vi "SetValueByArrayName.vi"(0 "VI Reference In":refnum<vi>, 2 "delimiter (>>)":string=">>", 5 "Control Path":string, 7 "Name Array":T1[](array[typedef]), 11 "Error In":errorcluster) -> (4 "VI Reference Out":refnum<vi>, 15 "Error Out":errorcluster)   [LabVIEW 2016, in "Drona.lvlib" / "ControlValue.lvlib" / "StimulusListbox.lvlib"]
doc: "Sets value(signaling) for the multi select listbox control whose item names with its occurrence are specified. Set the value as 1 in occurrence to select the first occurrence of an item. \n\nThe input control name is given as a string , incase of path, use delimiters inbetween the path."
uses:
  StimulusListbox.lvlib
  typedef/Name&Occurrence.ctl
  <userlib>/_OpenG.lib/array/array.llb/Search 1D Array (String)__ogtk.vi
  <vilib>/Utility/error.llb/Error Cluster From Error Code.vi
  <vilib>/ErrorRing/Error Ring.xnode
  Drona.lvlib
  Get/GetControlRef/GetControlRef.lvlib
  ControlValue.lvlib
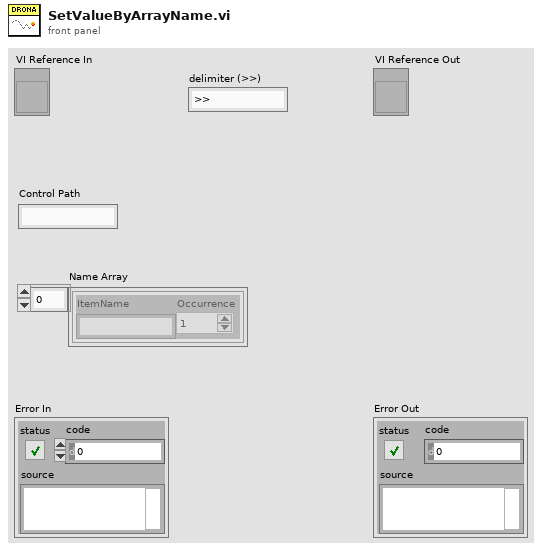
[diagram p1: front panel]
types:
  T1 = typedef "Drona.lvlib/ControlValue.lvlib/Name&Occurrence.ctl" = cluster{"ItemName":string, "Occurrence":i32}
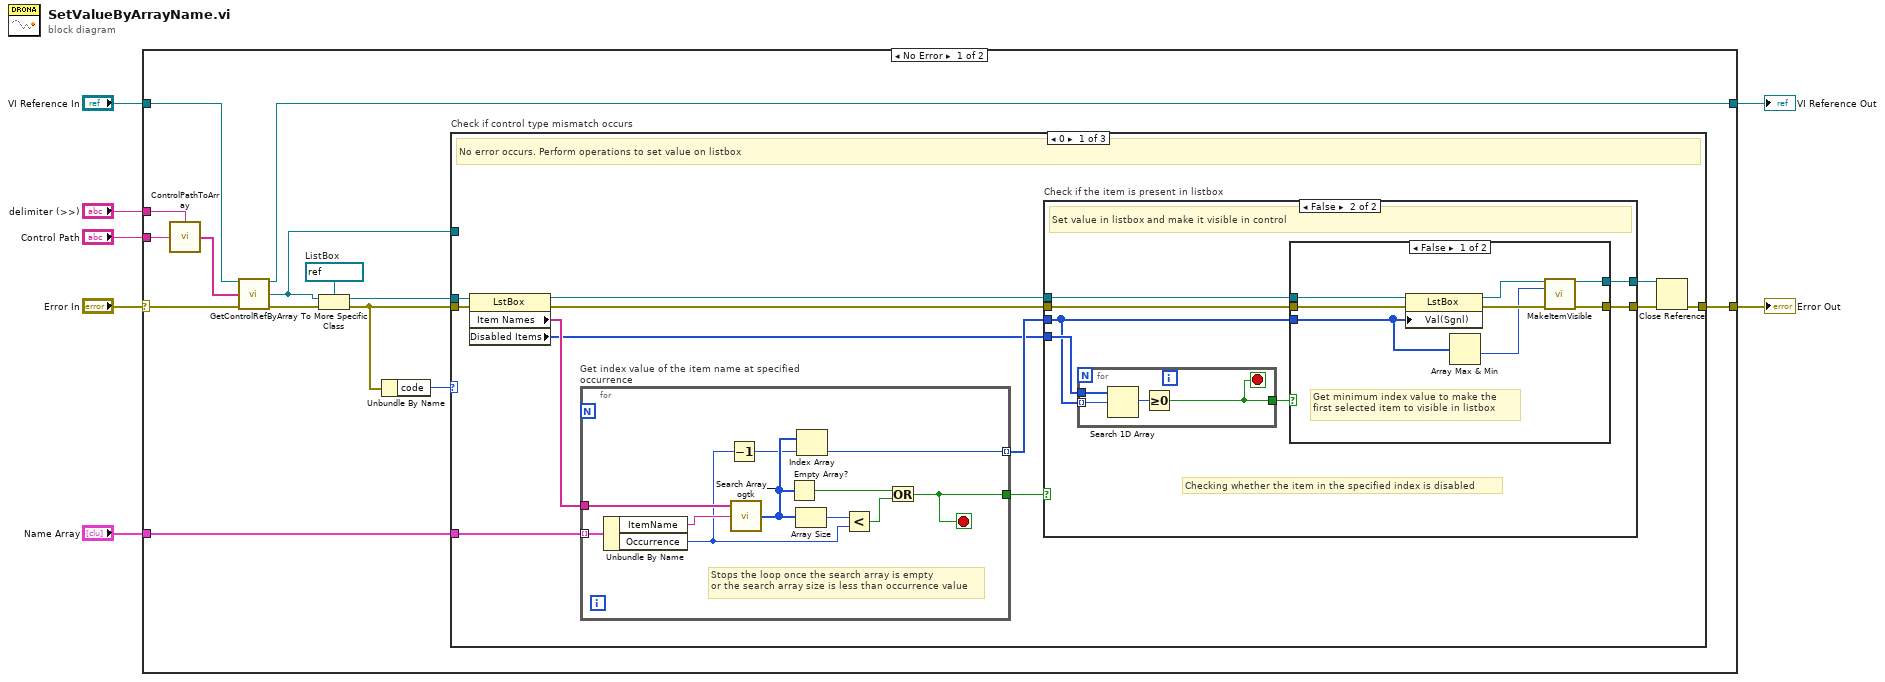
[diagram p0: block diagram]
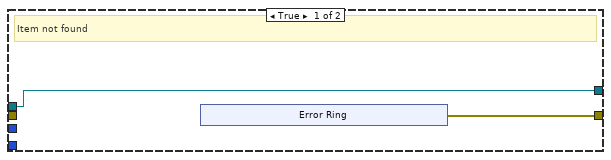
[diagram p2: hidden frame]
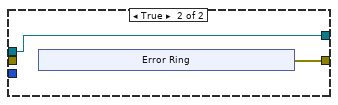
[diagram p3: hidden frame]
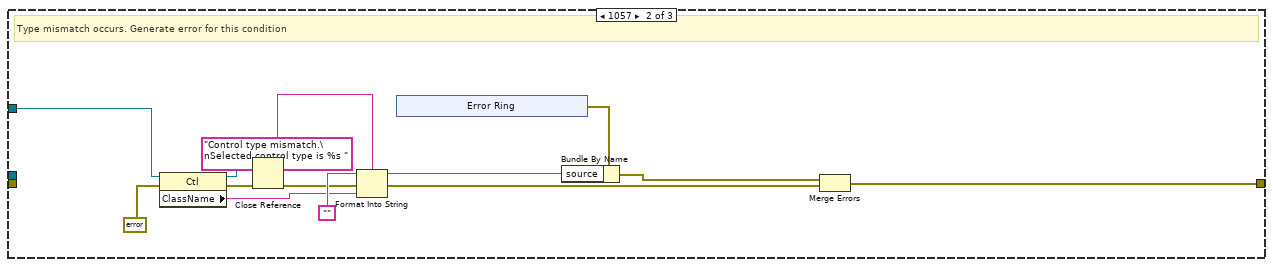
[diagram p4: hidden frame]
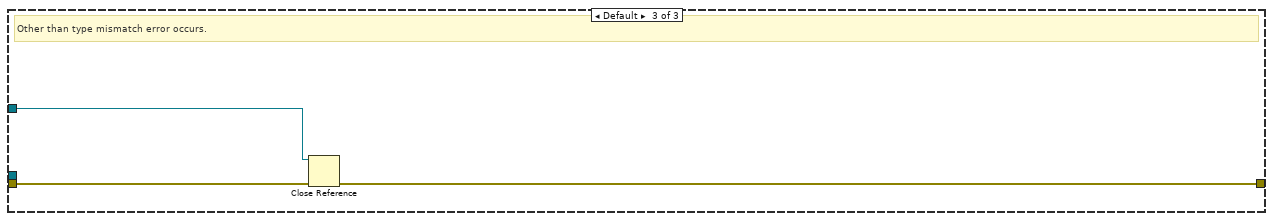
[diagram p5: hidden frame]
diagram:
  n1 = case shown="No Error" "Error In" {
    selector: "Error In" -> [w16 w100]
    tunnel: [w17 w100] -> w6
    tunnel: "VI Reference In" -> [w15 w99]
    tunnel: "Control Path" -> [w19 _]
    tunnel: [w12 w99] -> w3
    tunnel: "delimiter (>>)" -> [w18 _]
    tunnel: "Name Array" -> [w11 _]
    frame No Error {
      w21 = refnum<vi> refnum  # ListBox
      n2 = call "ControlPathToArray.vi"("Control Name"=w19, "delimiter (>>)"=w18) -> ("Control Path"=w14:string[])
      n3 = call "GetControlRefByArray.vi"("VI Reference In"=w15, "Control Path"=w14, "error In"=w16) -> ("VI Reference Out"=w12:refnum<vi>, "Ctl Refnum"=w8:refnum<vi>, "error out"=w13:errorcluster)  [unwired: 10 in]
      n4 = To More Specific Class(target class=w21, reference=w8, error in=w13) -> (specific class reference=w20:refnum<vi>, error out=w10:errorcluster)
      n5 = Unbundle By Name(w10) -> ("code"=w9:i32)
      n6 = case "Check if control type mismatch occurs" shown="0" w9 {
        tunnel: w10 -> [w33 _ w98]
        tunnel: w20 -> [w32 _ _]
        tunnel: [w31 w78 w97] -> w17
        tunnel: w11 -> [w27 _ _]
        tunnel: w8 -> [_ w79 w96]
        frame 0 {
          # "No error occurs. Perform operations to set value on listbox"
          n7 = property class="LstBox"(reference=w32, error in=w33) -> (reference out=w25:refnum<vi>, error out=w26:errorcluster, "Item Names"=w30:string[], "Disabled Items"=w22:i32[])
          n8 = for "Get index value of the item name at specified occurrence" {
            tunnel: w30 -> [w43]
            tunnel: w27 -> [w44] mode=indexing
            tunnel: [w35] -> w24 mode=indexing
            tunnel: [w34] -> w23
            stop <- w34 stop-if-true
            # "Stops the loop once the search array is empty \nor the search array size is less than occurrence value"
            n9 = Unbundle By Name(w44) -> ("ItemName"=w42:string, "Occurrence"=w37:i32)
            n10 = Decrement(x=w37) -> (x-1=w36:i32)
            n11 = call-poly <userlib>:"Search Array__ogtk.vi"("Array"=w43, "Element Data"=w42) -> ("Indices of Elements"=w38:i32[])  [unwired: 7 in]
            n12 = Empty Array?(array=w38) -> (empty?=w39:bool)
            n13 = Array Size(array=w38) -> (size(s)=w41:i32)
            n14 = Index Array(array=w38, index=w36) -> (element=w35:i32)
            n15 = Less?(x=w41, y=w37) -> (x < y?=w40:bool)
            n16 = Or(x=w39, y=w40) -> (x .or. y?=w34:bool)
          }
          n17 = case "Check if the item is present in listbox" shown="False" w23 {
            tunnel: [w46 w58] -> w29
            tunnel: [w45 w57] -> w28
            tunnel: w26 -> [_ w56]
            tunnel: w25 -> [w45 w55]
            tunnel: w24 -> [_ w52]
            tunnel: w22 -> [_ w53]
            frame True {
              # "Item not found"
              n18 = xnode "Error Ring"() -> ("error out"=w46:errorcluster)
            }
            frame False {
              # "Checking whether the item in the specified index is disabled"
              # "Set value in listbox and make it visible in control"
              n19 = for {
                tunnel: w52 -> [w61] mode=indexing
                tunnel: w53 -> [w62]
                tunnel: [w59] -> w54
                stop <- w59 stop-if-true
                n20 = Search 1D Array(1D array=w62, element=w61) -> (index of element=w60:i32)  [unwired: 1 in]
                n21 = Greater Or Equal To 0?(x=w60) -> (x >= 0?=w59:bool)
              }
              n22 = case shown="False" w54 {
                tunnel: [w69 w71] -> w58
                tunnel: [w67 w72] -> w57
                tunnel: w56 -> [w65 _]
                tunnel: w55 -> [w64 w72]
                tunnel: w52 -> [w63 _]
                frame False {
                  # "Get minimum index value to make the \nfirst selected item to visible in listbox"
                  n23 = property class="LstBox"(reference=w64, error in=w65, "Val(Sgnl)"=w63) -> (reference out=w68:refnum<vi>, error out=w70:errorcluster)
                  n24 = Array Max & Min(array=w63) -> (min value=w66:i32)  [unwired: 3 out]
                  n25 = call "MakeItemVisible.vi"("ListBox Ref In"=w68, "Item Index"=w66, "Error In"=w70) -> ("ListBox Ref Out"=w67:refnum<vi>, "Error Out"=w69:errorcluster)  [unwired: 11 in]
                }
                frame True {
                  n26 = xnode "Error Ring"() -> ("error out"=w71:errorcluster)
                }
              }
            }
          }
          n27 = Close Reference(reference=w28, error in (no error)=w29) -> (error out=w31:errorcluster)
        }
        frame 1057 {
          # "Type mismatch occurs. Generate error for this condition"
          n28 = property class="Ctl"(reference=w79, error in=errorcluster {"status"=FALSE, "code"=0, "source"=""} ("error out")) -> (reference out=w80:refnum<vi>, error out=w90:errorcluster, "ClassName"=w87:string)
          n29 = Close Reference(reference=w80, error in (no error)=w90) -> (error out=w81:errorcluster)
          n30 = Format Into String(format string="Control type mismatch.\nSelected control type is %s ", initial string="", error in=w81, w87) -> (resulting string=w84:string, error out=w82:errorcluster)
          n31 = xnode "Error Ring"() -> ("error out"=w85:errorcluster)
          n32 = Bundle By Name(cluster=w85, "source"=w84) -> (w83:errorcluster)
          n33 = Merge Errors(w83, w82) -> (w78:errorcluster)
        }
        frame Default {
          # "Other than type mismatch error occurs."
          n34 = Close Reference(reference=w96, error in (no error)=w98) -> (error out=w97:errorcluster)
        }
      }
    }
    frame Error {
    }
  }
  "Error Out" <- w6
  "VI Reference Out" <- w3
